vi "TDMS_RotateIfFull.vi"(8 "error in (no error)":errorcluster, 10 "state in":T1={"ref TDMS"=refnum, "File Path"=path "", "counter"=0, "Folder tmp"=path "/home/lvuser/lab9data/tmp", "folder ready"=path "/home/lvuser/lab9data/ready"}, 11 "max samples":i32) -> (0 "error out":errorcluster, 3 "state out":T1)   [LabVIEW 2025]
uses:
  Logger_State.ctl
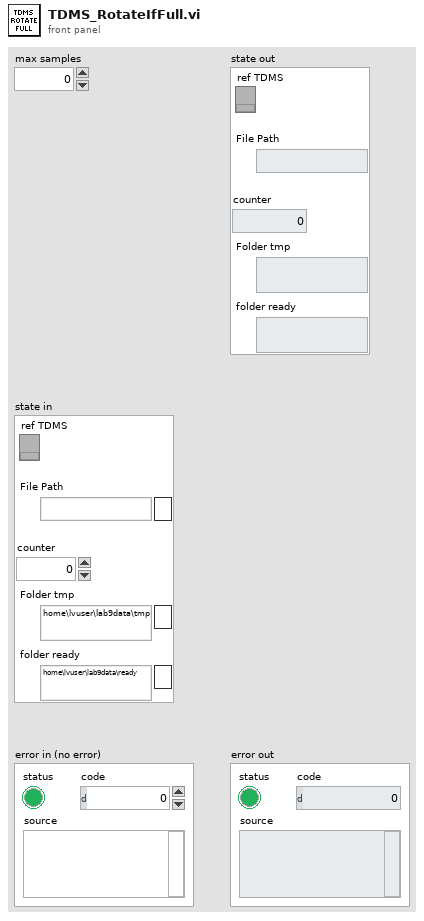
[diagram p1: front panel]
types:
  T1 = typedef "Logger_State.ctl" = cluster{"ref TDMS":refnum<k34>, "File Path":path, "counter":i32, "Folder tmp":path, "folder ready":path}
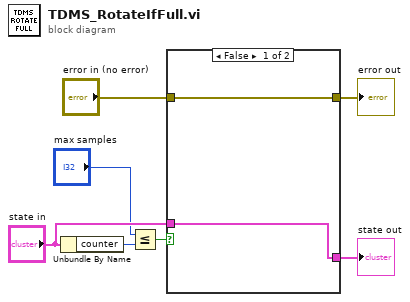
[diagram p0: block diagram]
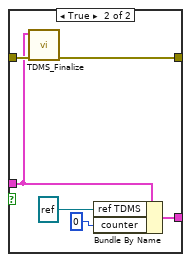
[diagram p2: hidden frame]
diagram:
  n1 = Unbundle By Name("state in") -> ("counter"=w1:i32)
  n2 = Less Or Equal?(x="max samples", y=w1) -> (x <= y?=w3:bool)
  n3 = case shown="False" w3 {
    tunnel: "state in" -> [w8 w13]
    tunnel: "error in (no error)" -> [w9 w15]
    tunnel: [w9 w14] -> w6
    tunnel: [w8 w10] -> w7
    frame False {
    }
    frame True {
      n4 = call "TDMS_Finalize.vi"("error in (no error)"=w15, "state in"=w13) -> ("error out"=w14:errorcluster)  [unwired: 9 in]
      n5 = Bundle By Name(cluster=w13, "ref TDMS"=refnum<k34> refnum, "counter"=0) -> (w10:T1)
    }
  }
  "error out" <- w6
  "state out" <- w7
